vi "2.2.vi"() -> ()   [LabVIEW 2026]
panel:
  out "SR-3":i32
  out "SR-2":i32
  out "SR-1":dbl
  out "Вузол":dbl
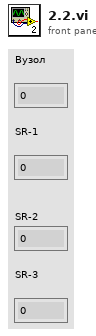
[diagram p1: front panel]
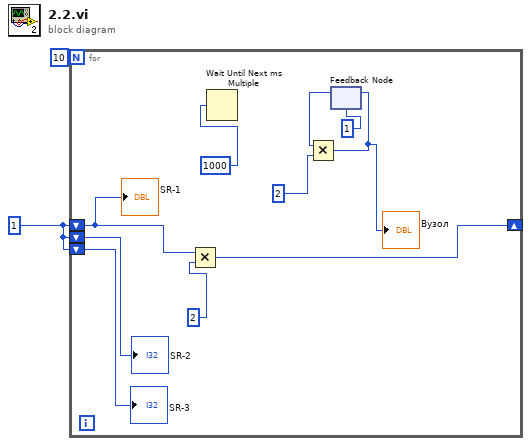
[diagram p0: block diagram]
diagram:
  w1 = 1
  n1 = for {
    N: 10 -> [_]
    shift-right: [w6] -> _
    shift-left: w1 -> [w5]
    shift-left: w1 -> [w4]
    shift-left: w1 -> [w3]
    n2 = Multiply(x=w5, y=2) -> (x*y=w6:i32)
    n3 = Wait Until Next ms Multiple(millisecond multiple=1000) -> ()  [unwired: 1 out]
    n4 = feedback #1(1) -> (w9:i32)
    n5 = Multiply(x=w9, y=2) -> (x*y=w10:i32)
    "Вузол" <- w10
    n6 = feedback-in #1(w10) -> ()
    "SR-1" <- w5
    "SR-2" <- w4
    "SR-3" <- w3
  }
